vi "UNITTEST-JSON-RPC-I32-Element.vi"(8 "error in (no error)":errorcluster) -> (0 "error out":errorcluster)   [LabVIEW 2019]
uses:
  <vilib>/numeric/Random Number (Range) U64.vi
  4c12f335-3af6-49f5-9257-0130b4f6318c.vi
  e861ad0b-bed5-4796-b07d-8449c8f87c08.vi
  <vilib>/numeric/sub_Random U32.vi
  JSON-RPC/API/JSON to Variant.vi
  <vilib>/Utility/Data Type/Get Type Information.vi
  <vilib>/JDP Science/JSONtext/JSON type.vi
  <vilib>/JDP Science/JSONtext/Get Array Elements.vi
  <vilib>/JDP Science/JSONtext/JSON text to Variant.vi
  <vilib>/addons/_JKI Toolkits/Caraya/classes/Assert/Assert Equal Value_Variant.vi
  <vilib>/addons/_JKI Toolkits/Caraya/classes/Assert/Assert Not Error.vi
  JSON-RPC/JSON-RPC.lvlib
  <vilib>/addons/_JKI Toolkits/Caraya/classes/Assert/Assert.lvclass
  <vilib>/addons/_JKI Toolkits/Caraya/classes/Test/Test.lvclass
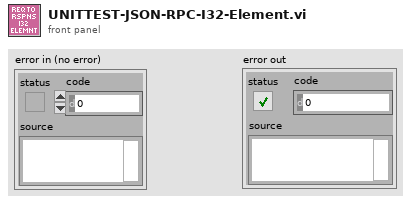
[diagram p1: front panel]
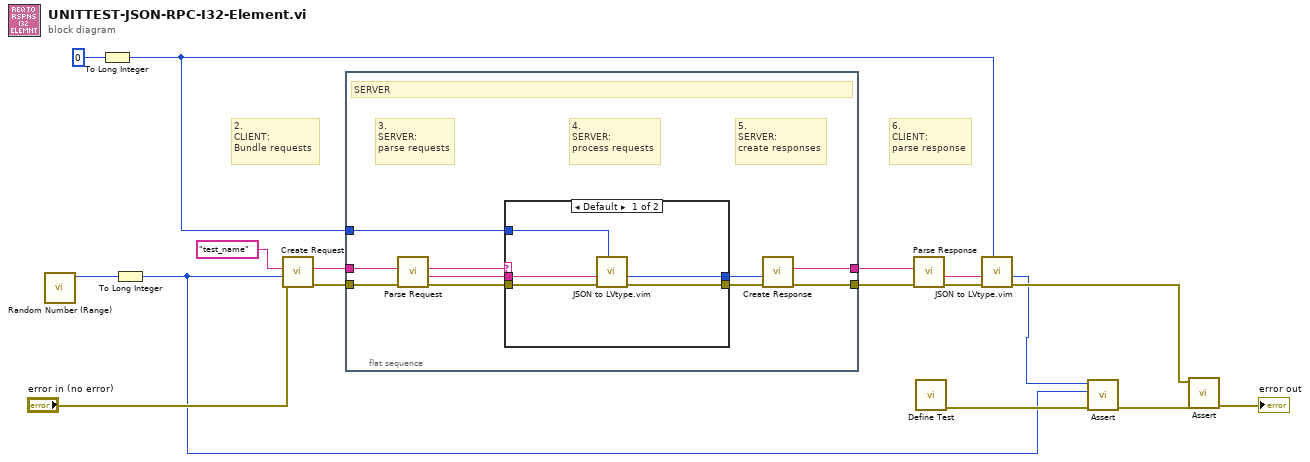
[diagram p0: block diagram]
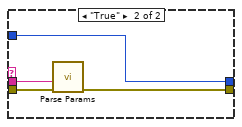
[diagram p2: hidden frame]
diagram:
  # "6.\nCLIENT:\nparse response"
  # "2.\nCLIENT:\nBundle requests"
  n1 = call-poly <vilib>:"Random Number (Range).vi"() -> ("number"=w4:u64)  [unwired: 11 in]
  n2 = To Long Integer(number=u64 0) -> (32bit integer=w2:i32)
  n3 = To Long Integer(number=w4) -> (32bit integer=w1:i32)
  n4 = call "Create Request.vi"("error in (no error)"="error in (no error)", "params"=w1, "method"="test_name") -> ("error out"=w16:errorcluster, "<JSON> Requests"=w17:string)  [unwired: 6 in, 1 out]
  n5 = flat-sequence {
    tunnel: w17 -> [w27]
    tunnel: w16 -> [w23]
    tunnel: [w22] -> w15
    tunnel: [w21] -> w14
    tunnel: w2 -> [w19]
    frame #0 {
      # "3.\nSERVER:\nparse requests"
      # "4.\nSERVER:\nprocess requests"
      # "5.\nSERVER:\ncreate responses"
      # "SERVER"
      n6 = call "Parse Request.vi"("error in (no error)"=w23, "<JSON> Requests"=w27) -> ("error out"=w24:errorcluster, "Params"=w25:string, "Methods"=w26:string)  [unwired: 6 in, 1 out]
      n7 = case shown="Default" w26 {
        tunnel: w25 -> [w29 w36]
        tunnel: w24 -> [w32 w35]
        tunnel: [w31 w34] -> w20
        tunnel: w19 -> [w30 w33]
        tunnel: [w28 w33] -> w18
        frame Default {
          n8 = call "JSON to LVtype.vim"("type"=w30, "error in (no error)"=w32, "JSON Data in"=w29) -> ("error out"=w31:errorcluster, "Data out"=w28:i32)  [unwired: 7 in]
        }
        frame "True" {
          n9 = call "Parse Params.vi"("error in (no error)"=w35, "<JSON> Params"=w36) -> ("error out"=w34:errorcluster)  [unwired: 7 in, 2 out]
        }
      }
      n10 = call "Create Response.vi"("error in (no error)"=w20, "result"=w18) -> ("error out"=w21:errorcluster, "<JSON> Response"=w22:string)  [unwired: 8 in]
    }
  }
  n11 = call "Parse Response.vi"("error in (no error)"=w14, "<JSON> Response"=w15) -> ("error out"=w13:errorcluster, "results"=w6:string)  [unwired: 7 in, 1 out]
  n12 = call <vilib>:"Define Test.vi"() -> ("error out"=w9:errorcluster)  [unwired: 10 in, 1 out]
  n13 = call "JSON to LVtype.vim"("type"=w2, "error in (no error)"=w13, "JSON Data in"=w6) -> ("error out"=w11:errorcluster, "Data out"=w3:i32)  [unwired: 7 in]
  n14 = call-poly <vilib>:"Assert.vi"("error in (no error)"=w9, "Actual"=w1, "Expected"=w3) -> ("error out"=w12:errorcluster)  [unwired: 7 in, 1 out]
  n15 = call-poly <vilib>:"Assert.vi"("error in (no error)"=w12, "Not Error?"=w11) -> ("error out"=→"error out":errorcluster)  [unwired: 8 in, 1 out]
